vi "_GetLineAngle.vi"(11 "Line":T1) -> (3 "Angle":dbl)   [LabVIEW 2020, in "OpenLvVision_Overlays.lvlib"]
uses:
  OpenLvVision_Overlays.lvlib
  TypeDefs/Line.ctl
  TypeDefs/PointI32.ctl
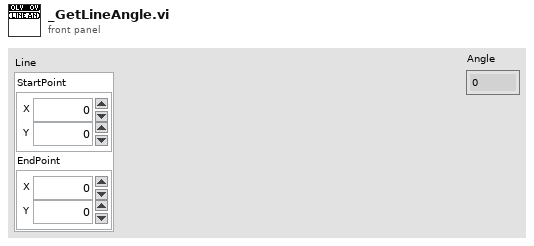
[diagram p1: front panel]
types:
  T1 = typedef "OpenLvVision_Overlays.lvlib/Line.ctl" = cluster{"StartPoint":T2, "EndPoint":T2}
  T2 = typedef "OpenLvVision_Overlays.lvlib/PointI32.ctl" = cluster{"X":i32, "Y":i32}
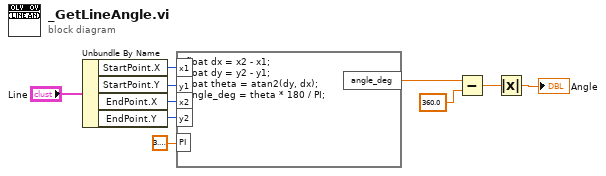
[diagram p0: block diagram]
diagram:
  n1 = Unbundle By Name("Line") -> ("StartPoint.X"=w8:i32, "StartPoint.Y"=w7:i32, "EndPoint.X"=w6:i32, "EndPoint.Y"=w5:i32)
  n2 = formula code="float dx = x2 - x1;\nfloat dy = y2 - y1;\nfloat theta = atan2(dy, dx);\nangle_deg = theta * 180 / PI;"("x1"=w8, "y1"=w7, "x2"=w6, "y2"=w5, "PI"=3.141592653589793) -> ("angle_deg"=w4:dbl)
  n3 = Subtract(x=w4, y=360.0) -> (x-y=w2:dbl)
  n4 = Absolute Value(x=w2) -> (abs(x)=→"Angle":dbl)
